vi "Channels.vi"() -> (2 "Names":string[](array[string]), 3 "Channels to Create":T1[](array[typedef]) {"Custom Config Data" format="%x"})   [LabVIEW 2021, in "CAN_Writer_CANsub_Common.lvlib"]
uses:
  CAN_Writer_CANsub_Common.lvlib
  <vilib>/CIF Foundation/CIF Core/Channels/ChannelRegistrar/typedef/Registered Channel Types.ctl
  <vilib>/CIF Foundation/CIF Core/Channels/ChannelRegistrar/ChannelRegistrar.lvlib
  <vilib>/CIF Foundation/CIF Channels Core/ChannelCommon/ChannelCommon.lvlib
  <vilib>/CIF Foundation/CIF LabVIEW Scripting/Update Enum/Update Enum.lvlib
  <vilib>/CIF Foundation/CIF Core/Channels/ChannelRegistrar/typedef/Channel Definition.ctl
  <vilib>/CIF Foundation/CIF Channels Core/ChannelCommon/typedef/FIFO Flags.ctl
  <vilib>/CIF Foundation/CIF Channels Core/ChannelCommon/typedef/New FIFO Config.ctl
  <vilib>/CIF Foundation/CIF Channels Core/ChannelCommon/typedef/Direction.ctl
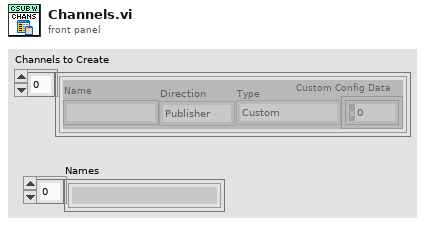
[diagram p1: front panel]
types:
  T1 = typedef "ChannelRegistrar.lvlib/Channel Definition.ctl" = cluster{"Name":string, "Direction":T2, "Type":T3, "Custom Config Data":u8[]}
  T2 = typedef "ChannelCommon.lvlib/Direction.ctl" = enum8{"Publisher", "Subscriber"}
  T3 = typedef "ChannelRegistrar.lvlib/Registered Channel Types.ctl" = enum8{"Custom", "Double_Tag", "I64_Tag", "U64_Tag", "U8_FIFO", "CAN_FIFO", "L2Enet_FIFO", "DAQ_FIFO", "Universal_FIFO", "String_Tag"}
  T4 = typedef "ChannelCommon.lvlib/New FIFO Config.ctl" = cluster{"Max Bytes/Msg":u64, "Max Msg/FIFO":u64, "FIFO Flags":T5}
  T5 = typedef "ChannelCommon.lvlib/FIFO Flags.ctl" = cluster{"Backpressure":bool}
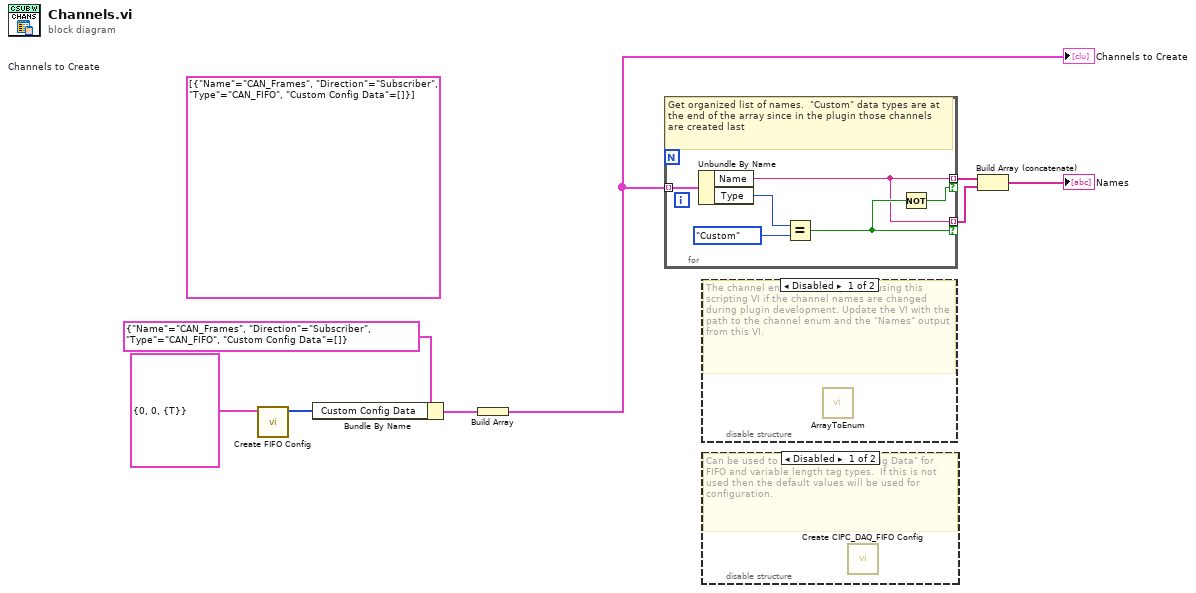
[diagram p0: block diagram]
diagram:
  (unwired) T1[] [{"Name"="CAN_Frames", "Direction"=enum."Subscriber", "Type"=enum."CAN_FIFO", "Custom Config Data"=[]}]  # Channels to Create
  n1 = call <vilib>:"Create FIFO Config.vi"("New FIFO Config"=T4 {"Max Bytes/Msg"=0, "Max Msg/FIFO"=0, "FIFO Flags"={"Backpressure"=TRUE}}) -> ("Flattened FIFO Config"=w3:u8[])  [unwired: 10 in]
  n2 = Bundle By Name(cluster=T1 {"Name"="CAN_Frames", "Direction"=enum."Subscriber", "Type"=enum."CAN_FIFO", "Custom Config Data"=[]} ("Channel Definition"), "Custom Config Data"=w3) -> (w2:T1)
  n3 = Build Array(w2) -> (w1:T1[])
  "Channels to Create" <- w1
  n4 = for {
    tunnel: w1 -> [w14] mode=indexing
    tunnel: [w9] -> w8 mode=indexing if=w10
    tunnel: [w9] -> w7 mode=indexing if=w11
    # "Get organized list of names.  \"Custom\" data types are at the end of the array since in the plugin those channels are created last"
    n5 = Unbundle By Name(w14) -> ("Name"=w9:string, "Type"=w13:T3)
    n6 = Equal?(x=w13, y=Registered_Channel_Types."Custom") -> (x = y?=w11:bool)
    n7 = Not(x=w11) -> (.not. x?=w10:bool)
  }
  n8 = disable-structure shown="Disabled" {
    frame Disabled {
      # "The channel enum can be updated using this scripting VI if the channel names are changed during plugin development. Update the VI with the path to the channel enum and the \"Names\" output from this VI."
      n9 = call <vilib>:"ArrayToEnum.vi"() -> ()  [unwired: 11 in, 1 out]
    }
    frame Enabled {
    }
  }
  n10 = disable-structure shown="Disabled" {
    frame Disabled {
      # "Can be used to create \"Custom Config Data\" for FIFO and variable length tag types.  If this is not used then the default values will be used for configuration."
      n11 = call <vilib>:"Create CIPC_DAQ_FIFO Config.vi"() -> ()  [unwired: 11 in, 1 out]
    }
    frame Enabled {
    }
  }
  n12 = Build Array (concatenate)(w8, w7) -> (→"Names":string[])
